vi "Concatenate.vi"() -> ()   [LabVIEW 2022 SP3]
panel:
  out "output array":dbl[](array[numeric])
  out "Array":dbl[][](array[numeric])
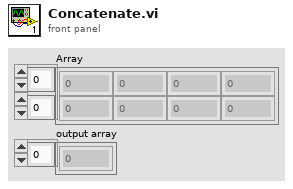
[diagram p1: front panel]
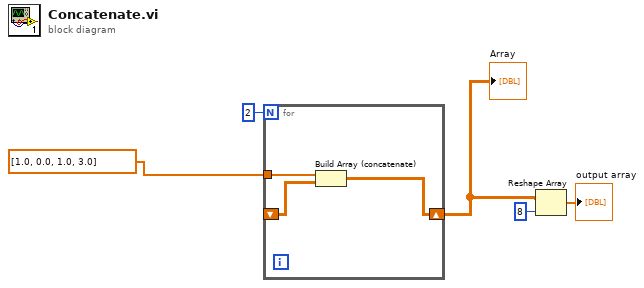
[diagram p0: block diagram]
diagram:
  n1 = for {
    N: 2 -> [_]
    shift-right: [w6] -> w3
    shift-left: _ -> [w8]
    tunnel: dbl[] [1.0, 0.0, 1.0, 3.0] ("bit array out") -> [w7]
    n2 = Build Array (concatenate)(w7, w8) -> (w6:dbl[][])
  }
  "Array" <- w3
  n3 = Reshape Array(w3, 8 ("dimension size")) -> (→"output array":dbl[])
